vi "Simplify Malleable Instance Name.vi"(8 "error in (no error)":errorcluster, 10 "Fully Qualified Malleable VI Name":string, 11 "Fully Qualified Malleable Instance Name":string) -> (0 "error out":errorcluster, 3 "Simple Malleable Instance Name":string)   [LabVIEW 2020, in "Peek Window.lvlib" / "Malleable VI Type.lvclass"]
uses:
  Malleable VI Type.lvclass
  <vilib>/regexp/Match Regular Expression.xnode
  Malleable VI Type.lvclass/Malleable VI Type.ctl
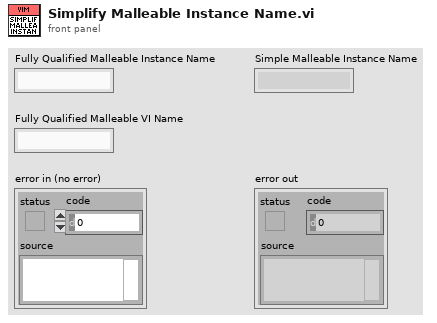
[diagram p1: front panel]
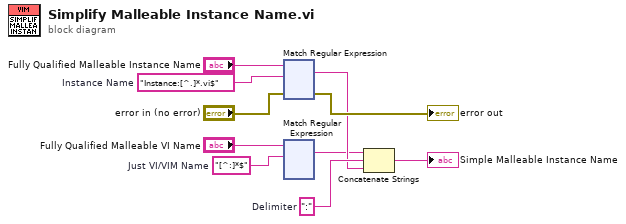
[diagram p0: block diagram]
diagram:
  w3 = "[^:]*$"  # Just VI/VIM Name
  w6 = ":"  # Delimiter
  w9 = "Instance:[^.]*.vi$"  # Instance Name
  n1 = xnode "Match Regular Expression"("input string"="Fully Qualified Malleable Instance Name", "regular expression"=w9, "error in"="error in (no error)") -> ("whole match"=w4:string, "error out"=→"error out":errorcluster)  [unwired: 3 in, 3 out]
  n2 = xnode "Match Regular Expression"("input string"="Fully Qualified Malleable VI Name", "regular expression"=w3) -> ("whole match"=w1:string)  [unwired: 4 in, 4 out]
  n3 = Concatenate Strings(w1, w6, w4) -> (→"Simple Malleable Instance Name":string)
